vi "RemoteVI Write Modifiers.vi"(0 "hWnd":u64, 1 "mods":u8, 11 "error in":errorcluster) -> (15 "error out":errorcluster)   [LabVIEW 2020, in "RemoteVI.lvlib"]
doc: "Writes the modifier keys the remote user holds into the key state of the UI thread that owns hWnd. A panel of this LabVIEW: RemoteVI Set Modifier Keys.vi (SetKeyboardState in this LabVIEW's UI thread). A window of another LabVIEW reached over VI Server (RemoteVI Remote Target.vi has an entry for hWnd): RemoteVI Remote Hooks.vi runs Set Modifier Keys INSIDE that process (RemoteVI Call Hooks.vi), so its UI thread gets them exactly as a panel of this LabVIEW does. Any other window (another process without VI Server): nothing is written - its key state belongs to its own input thread; the mouse messages still carry MK_SHIFT and MK_CONTROL. An incoming error skips the write."
uses:
  RemoteVI.lvlib
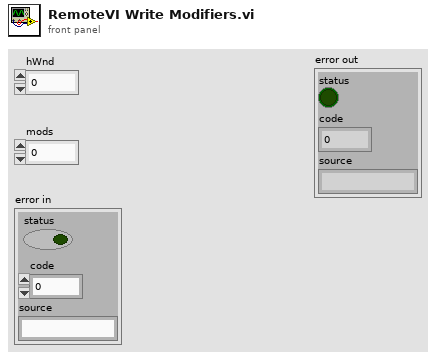
[diagram p1: front panel]
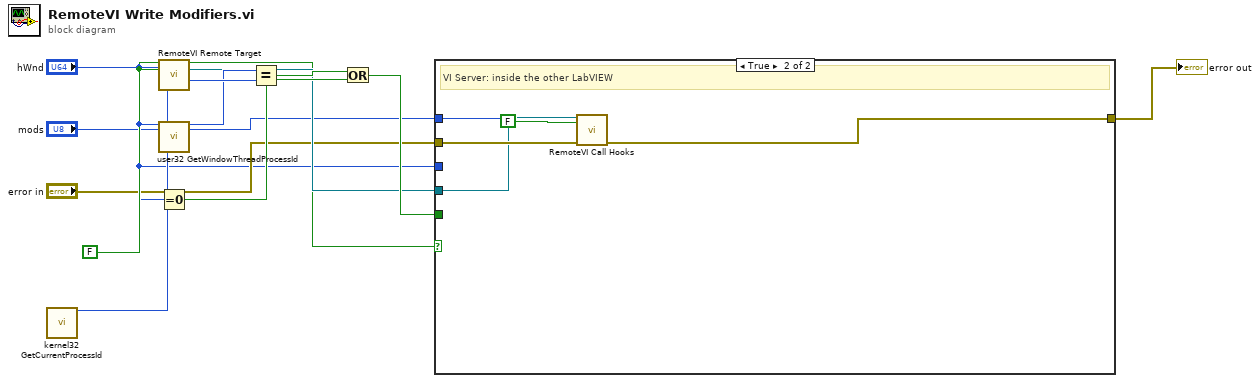
[diagram p0: block diagram]
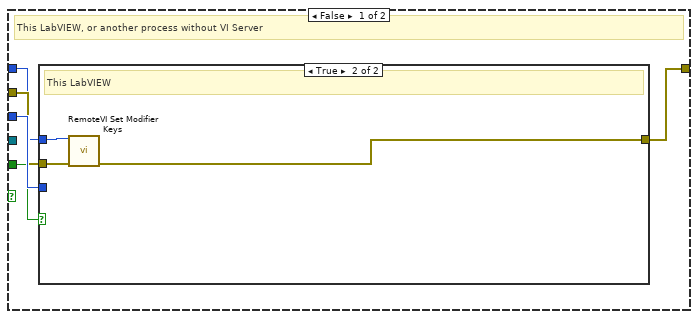
[diagram p2: hidden frame]
diagram:
  w4 = FALSE
  n1 = call "kernel32 GetCurrentProcessId.vi"() -> ("process ID"=w8:u32)  [unwired: 14 in, 1 out]
  n2 = call "RemoteVI Remote Target.vi"("put?"=w4, "hWnd"="hWnd", "remove?"=w4) -> ("found?"=w5:bool, "hooks out"=w6:refnum<vi>)  [unwired: 10 in, 1 out]
  n3 = call "user32 GetWindowThreadProcessId.vi"("hWnd"="hWnd") -> ("process ID"=w7:u32)  [unwired: 12 in, 2 out]
  n4 = Equal To 0?(x="hWnd") -> (x = 0?=w10:bool)
  n5 = Equal?(x=w7, y=w8) -> (x = y?=w9:bool)
  n6 = Or(x=w9, y=w10) -> (x .or. y?=w11:bool)
  n7 = case shown="True" w5 {
    tunnel: "mods" -> [w13 w23]
    tunnel: "error in" -> [w14 w24]
    tunnel: "hWnd" -> [w16 _]
    tunnel: w6 -> [_ w22]
    tunnel: w11 -> [w15 _]
    tunnel: [w17 w26] -> w12
    frame False {
      # "This LabVIEW, or another process without VI Server"
      n8 = case shown="True" w15 {
        tunnel: w13 -> [_ w19]
        tunnel: w14 -> [w18 w20]
        tunnel: w16 -> [_ _]
        tunnel: [w18 w21] -> w17
        frame False {
          # "Another process without VI Server: its key state cannot be set (only the mouse messages carry MK_SHIFT and MK_CONTROL)"
        }
        frame True {
          # "This LabVIEW"
          n9 = call "RemoteVI Set Modifier Keys.vi"("mods"=w19, "error in"=w20) -> ("error out"=w21:errorcluster)  [unwired: 13 in]
        }
      }
    }
    frame True {
      # "VI Server: inside the other LabVIEW"
      n10 = call "RemoteVI Call Hooks.vi"("hooks"=w22, "panel?"=FALSE, "mods"=w23, "error in"=w24) -> ("error out"=w26:errorcluster)  [unwired: 8 in, 3 out]
    }
  }
  "error out" <- w12
